vi "Reset Branch Status.vi"(8 "error in (no error)":errorcluster, 11 "bt_Parallel in":refnum<class "bt_Parallel.lvclass">) -> (0 "error out":errorcluster, 3 "bt_Parallel out":refnum<class "bt_Parallel.lvclass">)   [LabVIEW 2021, in "BT.lvlib" / "bt_Parallel.lvclass"]
uses:
  bt_Parallel.lvclass
  C:/Users/Tim/Documents/GitHub/LV_Behaviour_Tree/Source/Support/Nodes/Composites/abs_Composite/bt_Composite.lvclass
  abs_Composite/bt_Composite.lvclass/bt_Composite.ctl
  bt_Parallel.lvclass/bt_Parallel.ctl
  abs_Node/Status.ctl
  abs_Composite/Properties/Write Index.vi
  abs_Node/bt_Node.lvclass
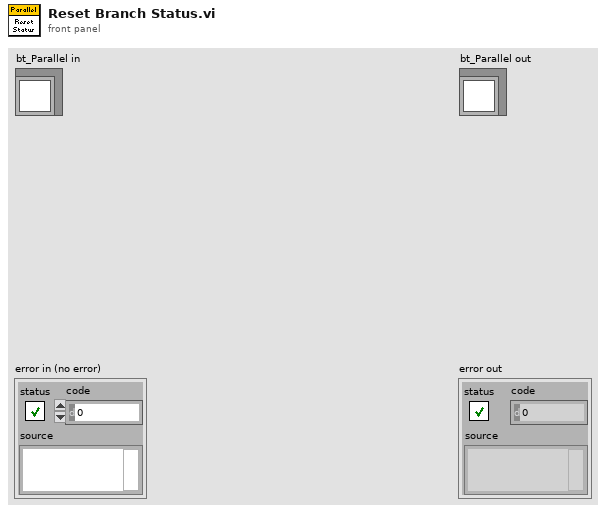
[diagram p1: front panel]
types:
  T1 = typedef "BT.lvlib/bt_Node.lvclass/Status.ctl" = enum16{"Success", "Failure", "Running"}
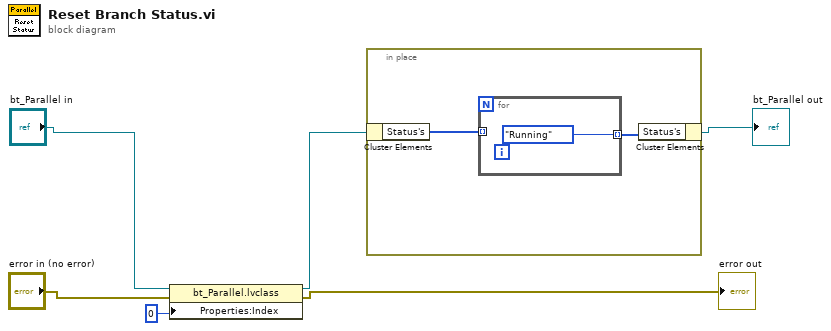
[diagram p0: block diagram]
diagram:
  n1 = property class="bt_Parallel.lvclass"(reference="bt_Parallel in", error in="error in (no error)", "Properties:Index"=0 ("Index")) -> (reference out=w3:refnum<class "bt_Parallel.lvclass">, error out=→"error out":errorcluster)
  n2 = in-place {
    n3 = in-place-cluster #1(w3) -> ("Status's"=w8:T1[])
    n4 = for {
      tunnel: w8 -> [_] mode=indexing
      tunnel: [Status."Running" ("Status")] -> w7 mode=indexing
    }
    n5 = in-place-cluster #1("Status's"=w7) -> (→"bt_Parallel out":refnum<class "bt_Parallel.lvclass">)
  }
